vi "strain__1822fcd108.vi"(8 "Gap":dbl, 9 "voltage to displacement contant":dbl, 10 "initial position in volt":dbl, 11 "displacement":dbl) -> (3 "strain":dbl)   [LabVIEW 2023]
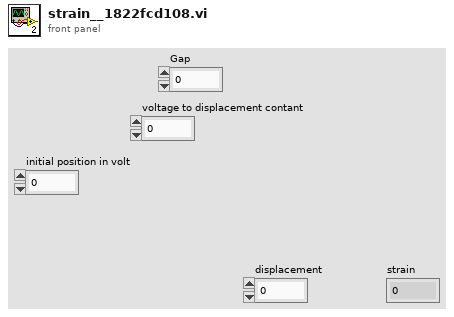
[diagram p1: front panel]
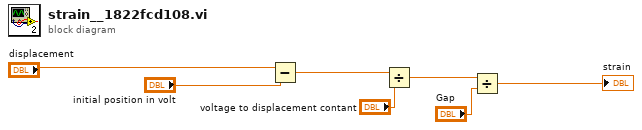
[diagram p0: block diagram]
diagram:
  n1 = Subtract(x="displacement", y="initial position in volt") -> (x-y=w7:dbl)
  n2 = Divide(x=w7, y="voltage to displacement contant") -> (x/y=w4:dbl)
  n3 = Divide(x=w4, y="Gap") -> (x/y=→"strain":dbl)
